vi "Write File.vi"(7 "Address":string, 8 "Error In":errorcluster) -> (0 "Error Out":errorcluster)   [LabVIEW 2018, in "Tests.lvlib" / "Known Hosts.lvlib"]
uses:
  Known Hosts.lvlib
  <vilib>/Utility/error.llb/Clear Errors.vi
  src/Toolkit/Known Hosts/Support/Create from Session.vi
  <vilib>/Utility/sysdir.llb/Get System Directory.vi
  src/Toolkit/Known Hosts/Support/Destroy to Session.vi
  <vilib>/addons/_JKI Toolkits/Caraya/classes/Test/Test.lvclass
  <vilib>/addons/_JKI Toolkits/Caraya/classes/Assert/Assert.lvclass
  src/Toolkit/Known Hosts/Known Hosts.lvclass
  Tests.lvlib
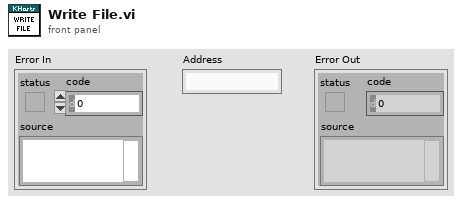
[diagram p1: front panel]
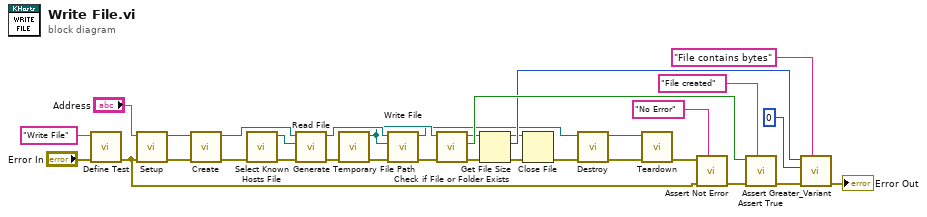
[diagram p0: block diagram]
diagram:
  n1 = call <vilib>:"Define Test.vi"("error in (no error)"="Error In", "Label (VI Title)"="Write File") -> ("error out"=w12:errorcluster)  [unwired: 9 in]
  n2 = call "Setup.vi"("Error In"=w12, "Address In"="Address") -> ("Error Out"=w7:errorcluster, "Sesssion"=w6:refnum<class "Session.lvclass">)  [unwired: 7 in, 1 out]
  n3 = call-poly "Create.vi"("Error In"=w7, "Session"=w6) -> ("Error Out"=w8:errorcluster, "Known Hosts"=w5:refnum<class "Known Hosts.lvclass">)  [unwired: 8 in]
  n4 = call "Select Known Hosts File.vi"("Error In"=w8) -> ("Error Out"=w30:errorcluster, "Known Hosts File"=w29:path)  [unwired: 9 in]
  n5 = call "Read File.vi"("Error In"=w30, "File"=w29, "Known Hosts In"=w5) -> ("Error Out"=w27:errorcluster, "Known Hosts Out"=w28:refnum<class "Known Hosts.lvclass">)  [unwired: 6 in, 1 out]
  n6 = call <vilib>:"Generate Temporary File Path.vi"("error in (no error)"=w27) -> ("error out"=w26:errorcluster, "Unique Temporary File Path"=w24:path)  [unwired: 9 in]
  n7 = call "Write File.vi"("Error In"=w26, "File"=w24, "Known Hosts In"=w28) -> ("Error Out"=w25:errorcluster, "Known Hosts Out"=w4:refnum<class "Known Hosts.lvclass">)  [unwired: 7 in]
  n8 = call <vilib>:"Check if File or Folder Exists.vi"("error in (no error)"=w25, "path"=w24) -> ("error out"=w18:errorcluster, "file or folder exists?"=w23:bool, "dup path"=w19:path)  [unwired: 7 in]
  n9 = Get File Size(file=w19, error in=w18) -> (refnum out=w3:refnum<file>, size (in bytes)=w15:i64, 0:w2:errorcluster)
  n10 = Close File(refnum=w3, error in=w2) -> (error out=w1:errorcluster)  [unwired: 1 out]
  n11 = call-poly "Destroy.vi"("Error In"=w1, "Known Hosts"=w4) -> ("Error Out"=w9:errorcluster, "Session"=w10:refnum<class "Session.lvclass">)  [unwired: 8 in]
  n12 = call "Teardown.vi"("Error In"=w9, "Session"=w10) -> ("Error Out"=w11:errorcluster)  [unwired: 9 in]
  n13 = call <vilib>:"Assert Not Error.vi"("Label"="No Error", "error in (no error)"=w12, "Not Error?"=w11) -> ("error out"=w22:errorcluster)  [unwired: 8 in]
  n14 = call <vilib>:"Assert True.vi"("Label"="File created", "error in (no error)"=w22, "True?"=w23) -> ("error out"=w21:errorcluster)  [unwired: 8 in]
  n15 = call <vilib>:"Assert Greater_Variant.vi"("Label"="File contains bytes", "error in (no error)"=w21, "Y"=i64 0 ("size (in bytes)"), "X"=w15) -> ("error out"=→"Error Out":errorcluster)  [unwired: 7 in]
